vi "Save VIs in a Folder.vi"(8 "error in (no error)":errorcluster, 11 "VI Folder":path) -> (0 "error out":errorcluster, 3 "VI List":path[](array[path]))   [LabVIEW 2016, in "SLL Scripting.lvlib"]
doc: "This VI can be used to save the list of all VIs in a folder."
uses:
  SLL Scripting.lvlib
panel:
  out "Progress":i32
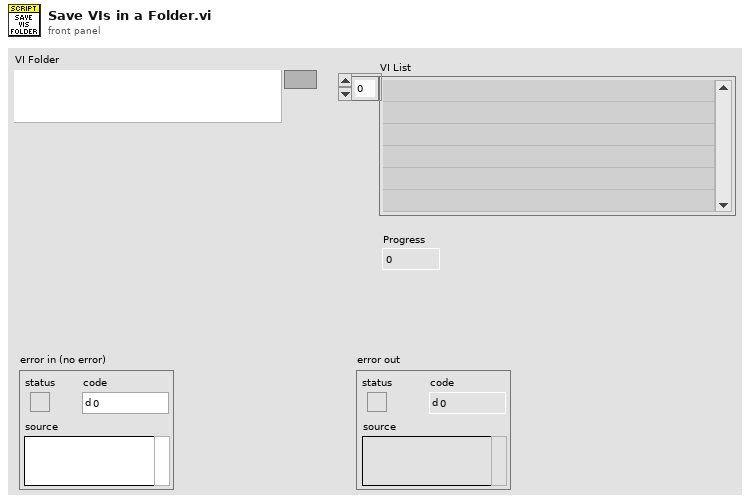
[diagram p1: front panel]
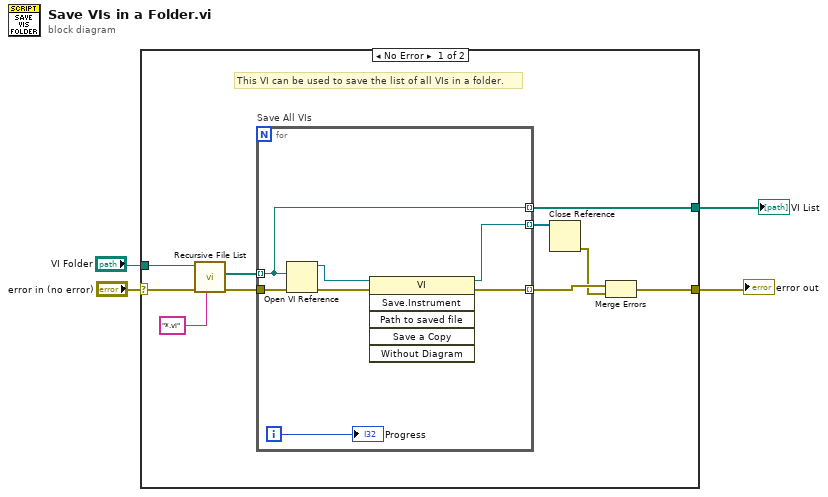
[diagram p0: block diagram]
diagram:
  n1 = case shown="No Error" "error in (no error)" {
    selector: "error in (no error)" -> [w9 w22]
    tunnel: "VI Folder" -> [w13 _]
    tunnel: [w10 _] -> w3
    tunnel: [w5 w22] -> w1
    frame No Error {
      # "This VI can be used to save the list of all VIs in a folder."
      n2 = call <vilib>:"Recursive File List.vi"("pattern"="*.vi", "error in (no error)"=w9, "Folder Path"=w13) -> ("error out"=w8:errorcluster, "All Files in Dir"=w11:path[])  [unwired: 4 in, 3 out]
      n3 = for "Save All VIs" {
        tunnel: [w15] -> w14 mode=indexing
        tunnel: w11 -> [w21] mode=indexing
        tunnel: [w21] -> w10 mode=indexing
        tunnel: w8 -> [w20]
        tunnel: [w17] -> w7 mode=indexing
        i -> [w18]
        n4 = Open VI Reference(vi path=w21, error in (no error)=w20) -> (vi reference=w16:refnum<vi>, error out=w19:errorcluster)  [unwired: 4 in]
        n5 = invoke class="VI" method="Save.Instrument"(reference=w16, error in=w19) -> (reference out=w15:refnum<vi>, error out=w17:errorcluster)  [unwired: 4 in, 4 out]
        "Progress" <- w18
      }
      n6 = Close Reference(reference=w14) -> (error out=w6:errorcluster)  [unwired: 1 in]
      n7 = Merge Errors(w7, w6) -> (w5:errorcluster)
    }
    frame Error {
    }
  }
  "error out" <- w1
  "VI List" <- w3
